vi "JsonRpcResponseStringToCluster.vi"(8 "error in (no error)":errorcluster, 10 "JsonRpcResponseJsonString":string) -> (0 "error out":errorcluster, 2 "JsonRPCHttpResponseBody":T1)   [LabVIEW 2017]
uses:
  <vilib>/LVH/i3 JSON/JSON Parsing/Get Object Parameter Files/Get Object Parameter - String.vi
  <vilib>/LVH/i3 JSON/JSON Parsing/Get Object Parameter Files/Get Object Parameter - Object.vi
  <vilib>/LVH/i3 JSON/JSON Parsing/Get Object Parameter Files/Get Object Parameter - Numeric.vi
  <vilib>/LVH/i3 JSON/i3-json.lvlib
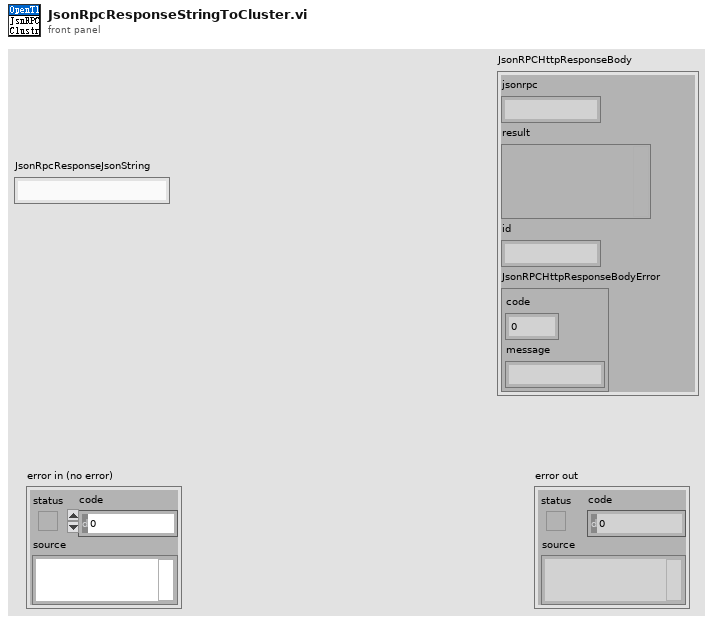
[diagram p1: front panel]
types:
  T1 = cluster{"jsonrpc":string, "result":variant, "id":string, "JsonRPCHttpResponseBodyError":cluster{"code":i32, "message":string}}
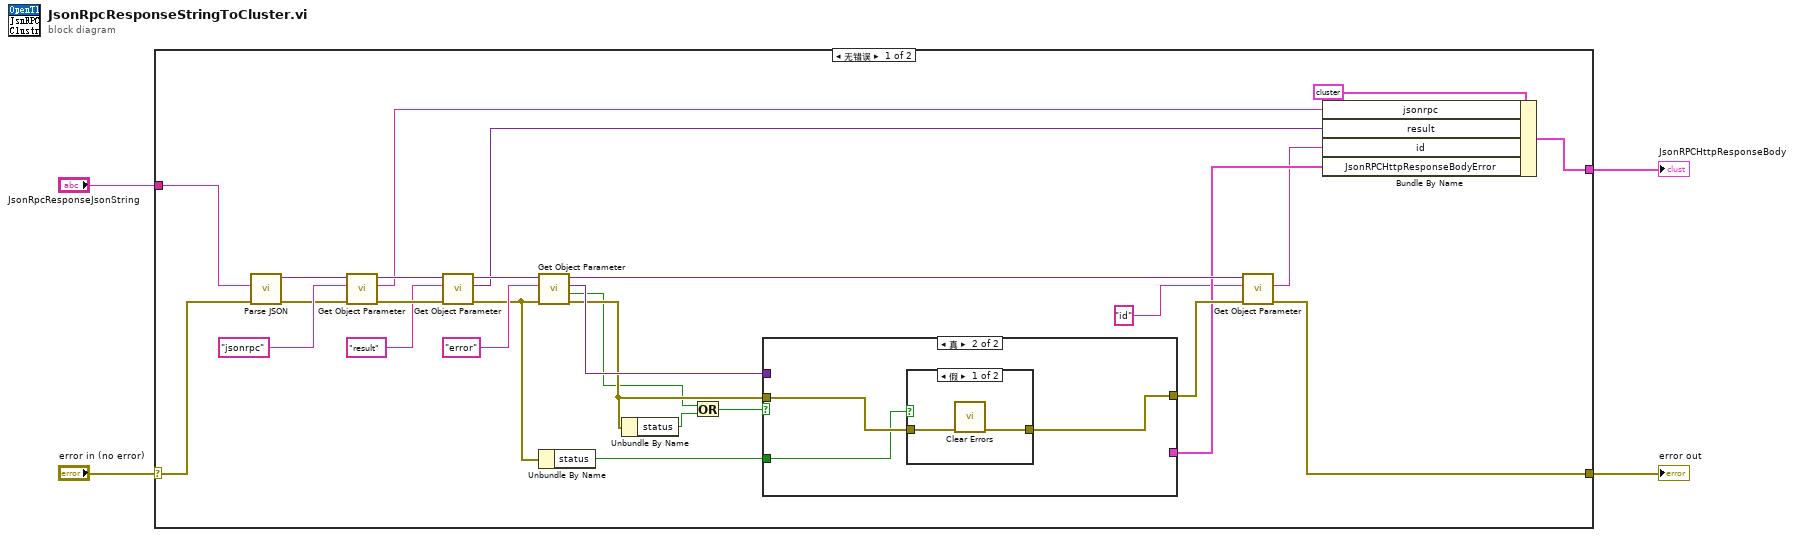
[diagram p0: block diagram]
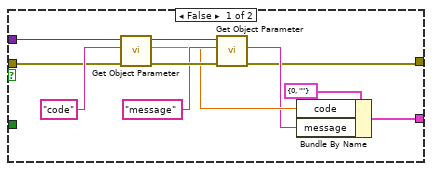
[diagram p2: hidden frame]
diagram:
  n1 = case shown="无错误" "error in (no error)" {
    selector: "error in (no error)" -> [w27 w49]
    tunnel: [w16 w49] -> w3
    tunnel: "JsonRpcResponseJsonString" -> [w31 _]
    tunnel: [w11 _] -> w1
    frame No Error {
      n2 = call <vilib>:"Parse JSON.vi"("error in (no error)"=w27, "JSON String"=w31) -> ("error out"=w28:errorcluster, "JSON Tree"=w29:variant)  [unwired: 6 in, 2 out]
      n3 = call-poly <vilib>:"Get Object Parameter.vi"("error in (no error)"=w28, "Parameter Name"="jsonrpc", "JSON Tree In (JSON Object)"=w29) -> ("error out"=w25:errorcluster, "String Value"=w15:string, "JSON Tree Out Passthrough"=w26:variant)  [unwired: 5 in, 1 out]
      n4 = call-poly <vilib>:"Get Object Parameter.vi"("error in (no error)"=w25, "Parameter Name"="result", "JSON Tree In (JSON Object)"=w26) -> ("error out"=w6:errorcluster, "JSON Object"=w14:variant, "JSON Tree Out Passthrough"=w24:variant)  [unwired: 5 in, 1 out]
      n5 = call-poly <vilib>:"Get Object Parameter.vi"("error in (no error)"=w6, "Parameter Name"="error", "JSON Tree In (JSON Object)"=w24) -> ("error out"=w10:errorcluster, "is JSON Null?"=w8:bool, "JSON Object"=w19:variant, "JSON Tree Out Passthrough"=w23:variant)  [unwired: 5 in]
      n6 = Unbundle By Name(w6) -> ("status"=w5:bool)
      n7 = Unbundle By Name(w10) -> ("status"=w9:bool)
      n8 = Or(x=w8, y=w9) -> (x .or. y?=w7:bool)
      n9 = case shown="真" w7 {
        tunnel: w19 -> [w37 _]
        tunnel: w10 -> [w34 w45]
        tunnel: [w33 w44] -> w18
        tunnel: [w32 _] -> w17
        tunnel: w5 -> [_ w43]
        frame False {
          n10 = call-poly <vilib>:"Get Object Parameter.vi"("error in (no error)"=w34, "Parameter Name"="code", "JSON Tree In (JSON Object)"=w37) -> ("error out"=w41:errorcluster, "Double Value"=w36:dbl, "JSON Tree Out Passthrough"=w40:variant)  [unwired: 5 in, 1 out]
          n11 = call-poly <vilib>:"Get Object Parameter.vi"("error in (no error)"=w41, "Parameter Name"="message", "JSON Tree In (JSON Object)"=w40) -> ("error out"=w33:errorcluster, "String Value"=w35:string)  [unwired: 5 in, 2 out]
          n12 = Bundle By Name(cluster=cluster{"code":i32, "message":string} {"code"=0, "message"=""} ("JsonRPCHttpResponseBodyError"), "code"=w36, "message"=w35) -> (w32:cluster{"code":i32, "message":string})
        }
        frame True {
          n13 = case shown="假" w43 {
            tunnel: w45 -> [w47 w48]
            tunnel: [w46 w48] -> w44
            frame False {
              n14 = call <vilib>:"Clear Errors.vi"("error in (no error)"=w47) -> ("error out"=w46:errorcluster)  [unwired: 5 in, 1 out]
            }
            frame True {
            }
          }
        }
      }
      n15 = call-poly <vilib>:"Get Object Parameter.vi"("error in (no error)"=w18, "Parameter Name"="id", "JSON Tree In (JSON Object)"=w23) -> ("error out"=w16:errorcluster, "String Value"=w12:string)  [unwired: 5 in, 2 out]
      n16 = Bundle By Name(cluster=T1 {"jsonrpc"="", "result"=variant, "id"="", "JsonRPCHttpResponseBodyError"={"code"=0, "message"=""}} ("JsonRPCHttpResponseBody"), "jsonrpc"=w15, "result"=w14, "id"=w12, "JsonRPCHttpResponseBodyError"=w17) -> (w11:T1)
    }
    frame Error {
    }
  }
  "error out" <- w3
  "JsonRPCHttpResponseBody" <- w1
